vi "LB_AssertIndexValue_Tests.vi"(11 "error in":errorcluster) -> (15 "error out":errorcluster)   [LabVIEW 2016, in "DronaTest.lvlib"]
uses:
  DronaTest.lvlib
  APIs/Stimulus/ControlValue/SetValueAuto.vi
  APIs/Assert/AssertControlValue/Controls/Listbox/AssertIndexValue.vi
  <vilib>/addons/_JKI Toolkits/Caraya/classes/Assert/Assert Error.vi
  <vilib>/addons/_JKI Toolkits/Caraya/classes/Assert/Assert Equal Value_Variant.vi
  <vilib>/addons/_JKI Toolkits/Caraya/classes/Test/Test.lvclass
  Drona.lvlib
  <vilib>/SLL Toolkit/SLL Debug/SLL Debug.lvlib
  <vilib>/addons/_JKI Toolkits/Caraya/classes/Assert/Assert.lvclass
  APIs/Assert/AssertControlValue/Controls/Listbox/AssertListbox.lvlib
  APIs/Stimulus/ControlValue/ControlValue.lvlib
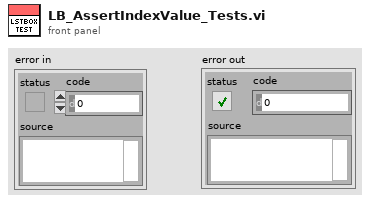
[diagram p1: front panel]
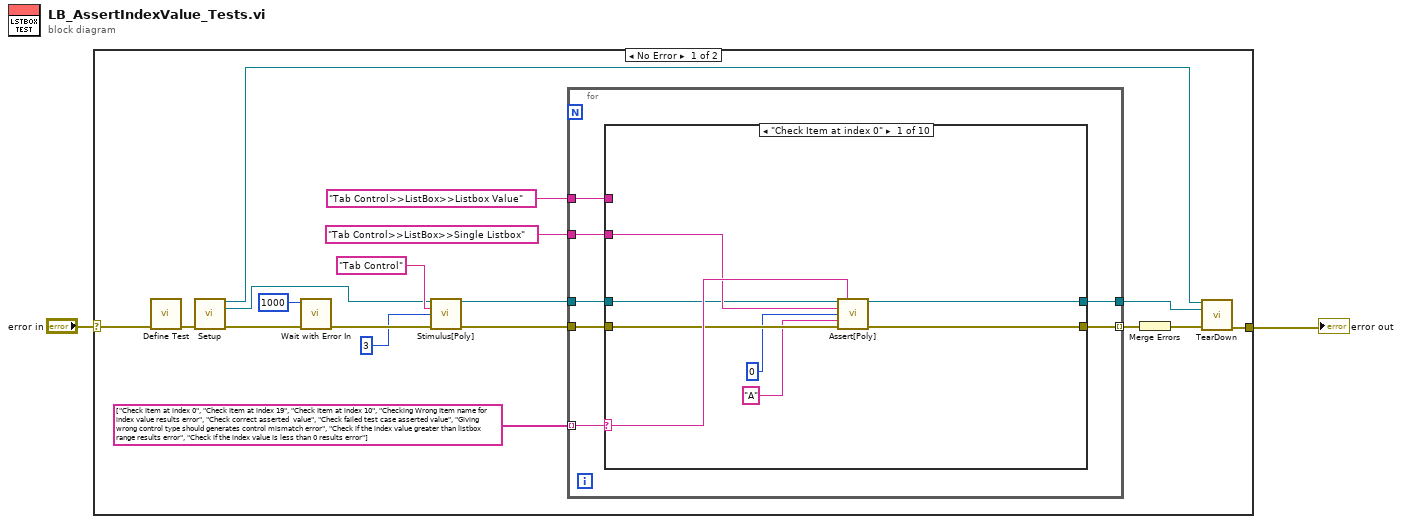
[diagram p0: block diagram]
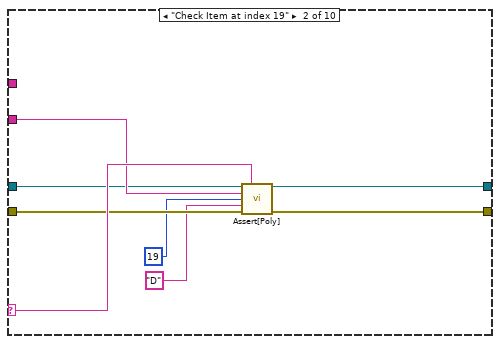
[diagram p2: hidden frame]
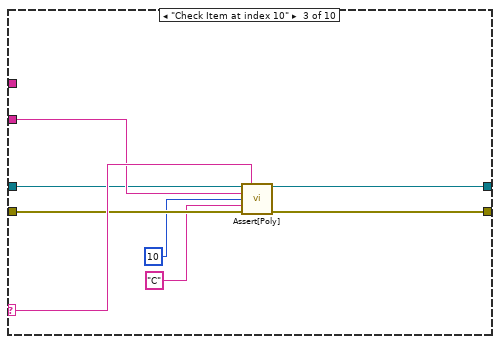
[diagram p3: hidden frame]
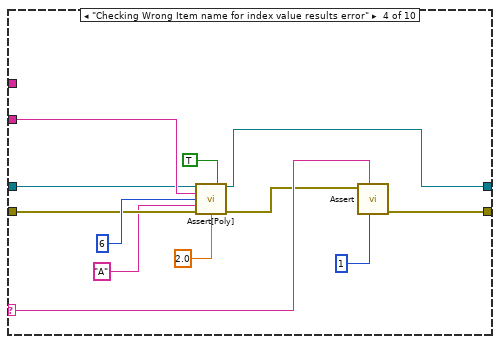
[diagram p4: hidden frame]
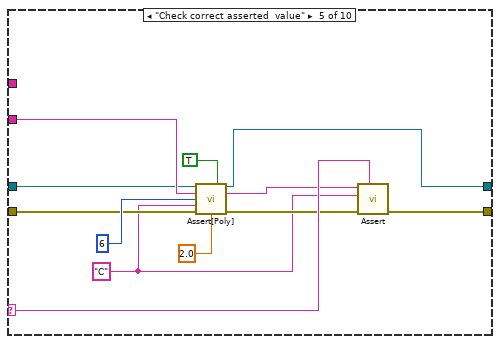
[diagram p5: hidden frame]
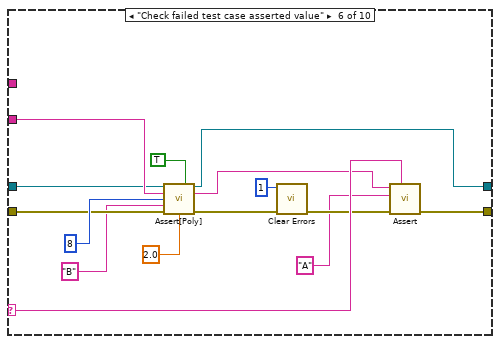
[diagram p6: hidden frame]
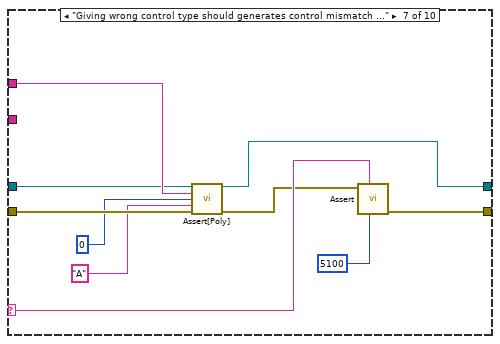
[diagram p7: hidden frame]
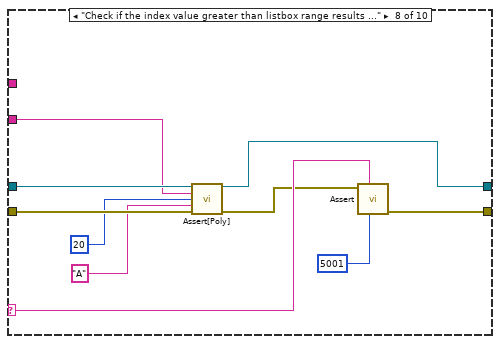
[diagram p8: hidden frame]
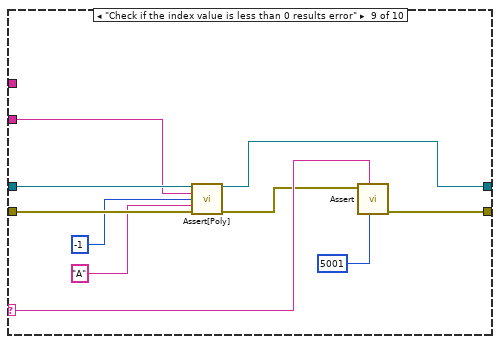
[diagram p9: hidden frame]
diagram:
  n1 = case shown="No Error" "error in" {
    selector: "error in" -> [w20 w123]
    tunnel: [w3 w123] -> w1
    frame No Error {
      n2 = call <vilib>:"Define Test.vi"("error in (no error)"=w20) -> ("error out"=w9:errorcluster)  [unwired: 9 in, 1 out]
      n3 = call "Setup.vi"("error in"=w9) -> ("Application Ref"=w5:refnum<vi>, "VI out"=w7:refnum<vi>, "error out"=w8:errorcluster)  [unwired: 12 in]
      n4 = call <vilib>:"Wait with Error In.vi"("error in (no error)"=w8, "milliseconds to wait"=u32 1000) -> ("error out"=w18:errorcluster)  [unwired: 9 in]
      n5 = call-poly "Stimulus[Poly].vi"("VI Reference In"=w7, "Control Path"="Tab Control", "Value (Signaling)"=3, "error in"=w18) -> ("VI Reference Out"=w14:refnum<vi>, "error out"=w17:errorcluster)  [unwired: 10 in]
      n6 = for {
        tunnel: w14 -> [w26]
        tunnel: "Tab Control>>ListBox>>Single Listbox" ("Control Path") -> [w25]
        tunnel: "Tab Control>>ListBox>>Listbox Value" ("Control Path") -> [w24]
        tunnel: string[] ["Check Item at index 0", "Check Item at index 19", "Check Item at index 10", "Checking Wrong Item name for index value results error", "Check correct asserted  value", "Check failed test case asserted value", "Giving wrong control type should generates control mismatch error", "Check if the index value greater than listbox range results error", "Check if the index value is less than 0 results error"] -> [w22] mode=indexing
        tunnel: [w21] -> w4
        tunnel: w17 -> [w27]
        tunnel: [w23] -> w10 mode=indexing
        n7 = case shown="\"Check Item at index 0\"" w22 {
          selector: w22 -> [w33 w41 w49 w62 w74 w89 w99 w109 w119 _]
          tunnel: w27 -> [w31 w39 w47 w54 w69 w84 w94 w105 w115 w122]
          tunnel: w26 -> [w30 w38 w46 w53 w68 w83 w93 w104 w114 w121]
          tunnel: w25 -> [w32 w40 w48 w60 w73 w88 _ w101 w111 _]
          tunnel: w24 -> [_ _ _ _ _ _ w96 _ _ _]
          tunnel: [w35 w43 w51 w63 w75 w90 w100 w110 w120 w122] -> w23
          tunnel: [w34 w42 w50 w58 w71 w86 w95 w106 w116 w121] -> w21
          frame "Check Item at index 0" {
            n8 = call-poly "Assert[Poly].vi"("VI Reference In"=w30, "Test Label"=w33, "Control Path"=w32, "Item Index"=0, "Item Value"="A", "Error In"=w31) -> ("VI Reference Out"=w34:refnum<vi>, "Error Out"=w35:errorcluster)  [unwired: 7 in, 1 out]
          }
          frame "Check Item at index 19" {
            n9 = call-poly "Assert[Poly].vi"("VI Reference In"=w38, "Test Label"=w41, "Control Path"=w40, "Item Index"=19, "Item Value"="D", "Error In"=w39) -> ("VI Reference Out"=w42:refnum<vi>, "Error Out"=w43:errorcluster)  [unwired: 7 in, 1 out]
          }
          frame "Check Item at index 10" {
            n10 = call-poly "Assert[Poly].vi"("VI Reference In"=w46, "Test Label"=w49, "Control Path"=w48, "Item Index"=10, "Item Value"="C", "Error In"=w47) -> ("VI Reference Out"=w50:refnum<vi>, "Error Out"=w51:errorcluster)  [unwired: 7 in, 1 out]
          }
          frame "Checking Wrong Item name for index value results error" {
            n11 = call-poly "Assert[Poly].vi"("VI Reference In"=w53, "Assert Only? (F)"=TRUE, "Control Path"=w60, "Item Index"=6, "Item Value"="A", "Error In"=w54, "Timeout(5 sec)"=2.0) -> ("VI Reference Out"=w58:refnum<vi>, "Error Out"=w57:errorcluster)  [unwired: 6 in, 1 out]
            n12 = call-poly <vilib>:"Assert.vi"("error code (1)"=1, "Label"=w62, "Error?"=w57) -> ("error out"=w63:errorcluster)  [unwired: 7 in, 1 out]
          }
          frame "Check correct asserted  value" {
            w65 = "C" ("Item Value")
            n13 = call-poly "Assert[Poly].vi"("VI Reference In"=w68, "Assert Only? (F)"=TRUE, "Control Path"=w73, "Item Index"=6, "Item Value"=w65, "Error In"=w69, "Timeout(5 sec)"=2.0) -> ("VI Reference Out"=w71:refnum<vi>, "Asserted Value"=w66:string, "Error Out"=w67:errorcluster)  [unwired: 6 in]
            n14 = call-poly <vilib>:"Assert.vi"("Label"=w74, "error in (no error)"=w67, "Y"=w65, "X"=w66) -> ("error out"=w75:errorcluster)  [unwired: 6 in, 1 out]
          }
          frame "Check failed test case asserted value" {
            n15 = call-poly "Assert[Poly].vi"("VI Reference In"=w83, "Assert Only? (F)"=TRUE, "Control Path"=w88, "Item Index"=8, "Item Value"="B", "Error In"=w84, "Timeout(5 sec)"=2.0) -> ("VI Reference Out"=w86:refnum<vi>, "Asserted Value"=w81:string, "Error Out"=w82:errorcluster)  [unwired: 6 in]
            n16 = call <vilib>:"Clear Errors.vi"("error in (no error)"=w82, "specific error code to clear (0: all)"=1) -> ("error out"=w79:errorcluster)  [unwired: 4 in, 1 out]
            n17 = call-poly <vilib>:"Assert.vi"("Label"=w89, "error in (no error)"=w79, "Y"="A" ("Item Value"), "X"=w81) -> ("error out"=w90:errorcluster)  [unwired: 6 in, 1 out]
          }
          frame "Giving wrong control type should generates control mismatch error" {
            n18 = call-poly "Assert[Poly].vi"("VI Reference In"=w93, "Control Path"=w96, "Item Index"=0, "Item Value"="A", "Error In"=w94) -> ("VI Reference Out"=w95:refnum<vi>, "Error Out"=w97:errorcluster)  [unwired: 8 in, 1 out]
            n19 = call-poly <vilib>:"Assert.vi"("error code (1)"=5100, "Label"=w99, "Error?"=w97) -> ("error out"=w100:errorcluster)  [unwired: 7 in, 1 out]
          }
          frame "Check if the index value greater than listbox range results error" {
            n20 = call-poly "Assert[Poly].vi"("VI Reference In"=w104, "Control Path"=w101, "Item Index"=20, "Item Value"="A", "Error In"=w105) -> ("VI Reference Out"=w106:refnum<vi>, "Error Out"=w107:errorcluster)  [unwired: 8 in, 1 out]
            n21 = call-poly <vilib>:"Assert.vi"("error code (1)"=5001, "Label"=w109, "Error?"=w107) -> ("error out"=w110:errorcluster)  [unwired: 7 in, 1 out]
          }
          frame "Check if the index value is less than 0 results error" {
            n22 = call-poly "Assert[Poly].vi"("VI Reference In"=w114, "Control Path"=w111, "Item Index"=-1, "Item Value"="A", "Error In"=w115) -> ("VI Reference Out"=w116:refnum<vi>, "Error Out"=w117:errorcluster)  [unwired: 8 in, 1 out]
            n23 = call-poly <vilib>:"Assert.vi"("error code (1)"=5001, "Label"=w119, "Error?"=w117) -> ("error out"=w120:errorcluster)  [unwired: 7 in, 1 out]
          }
          frame Default {
          }
        }
      }
      n24 = Merge Errors(w10) -> (w6:errorcluster)
      n25 = call "TearDown.vi"("Application Ref"=w5, "VI in"=w4, "error in (no error)"=w6) -> ("error out"=w3:errorcluster)  [unwired: 12 in]
    }
    frame Error {
    }
  }
  "error out" <- w1
